vi "Calculate Curve Distance.vi"(9 "error in (no error)":errorcluster, 11 "Points":T1[](array[typedef])) -> (1 "error out":errorcluster, 2 "Length":dbl, 3 "Points Out":T1[](array[typedef]), 5 "Distance vs t":cluster{"t":dbl[], "Distance":dbl[]})   [LabVIEW 2019, in "Tool Path.lvclass"]
uses:
  Tool Path.lvclass
  Parse/PathCommands/Point.ctl
  Parse/PathCommands/PathCommands.lvclass
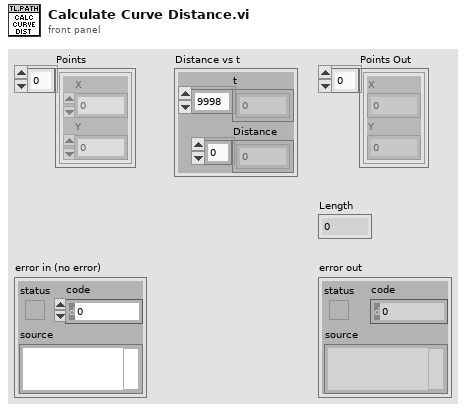
[diagram p1: front panel]
types:
  T1 = typedef "PathCommands.lvclass/Point.ctl" = cluster{"X":dbl, "Y":dbl}
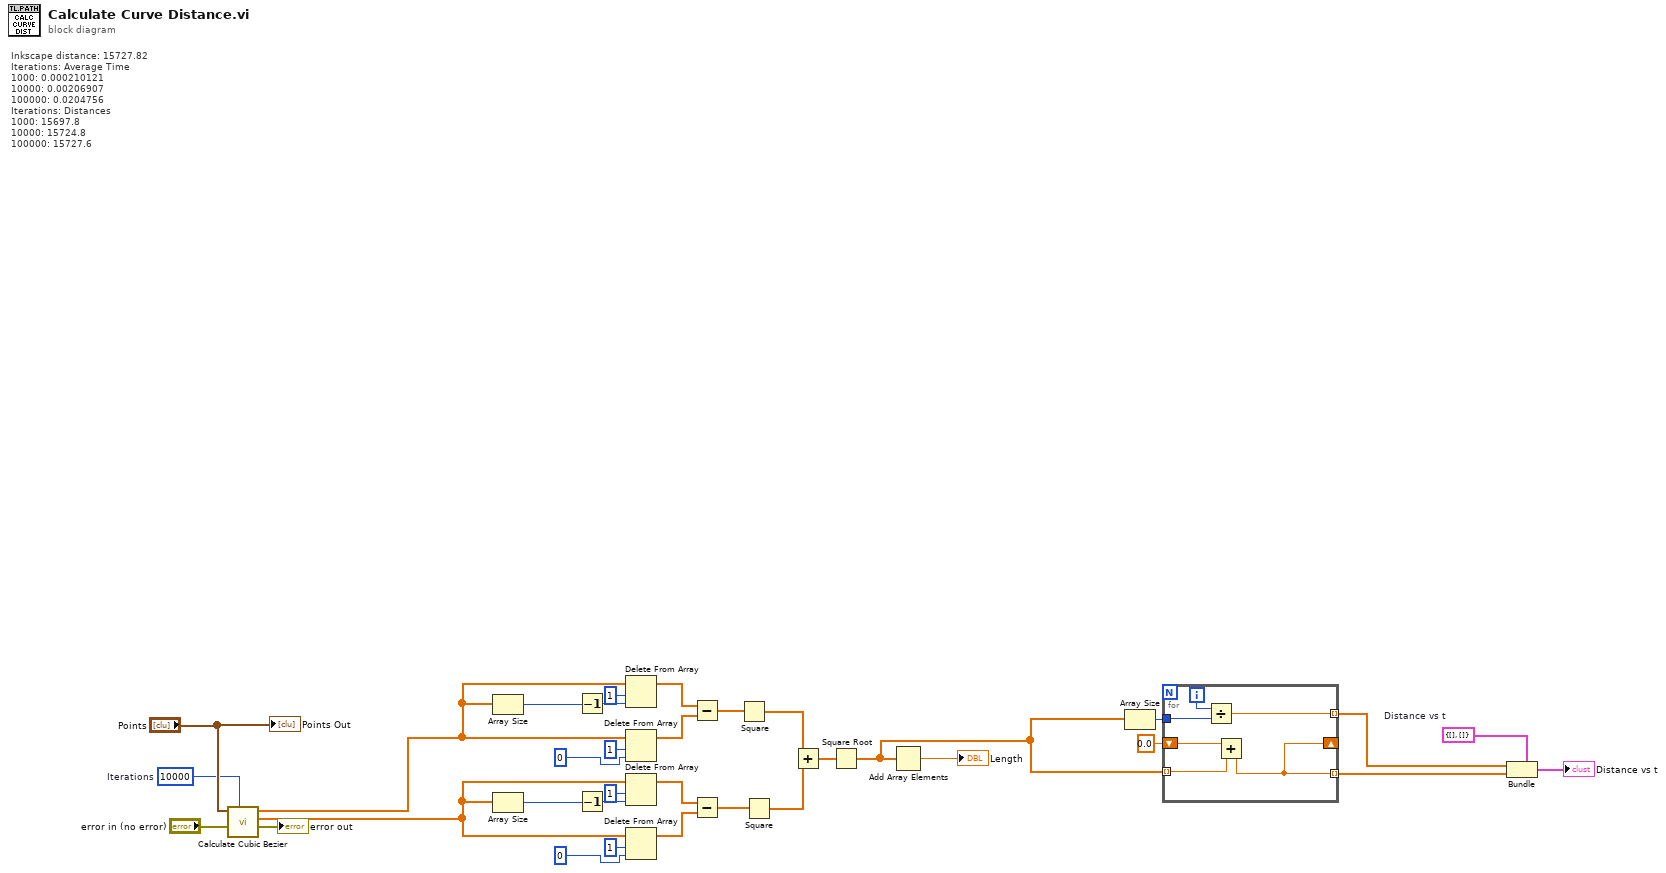
[diagram p0: block diagram]
diagram:
  w2 = cluster{"t":dbl[], "Distance":dbl[]} {"t"=[], "Distance"=[]}  # Distance vs t
  w27 = 10000  # Iterations
  # "Inkscape distance: 15727.82\nIterations: Average Time\n1000: 0.000210121\n10000: 0.00206907\n100000: 0.0204756\nIterations: Distances\n1000: 15697.8\n10000: 15724.8\n100000: 15727.6"
  n1 = call "Calculate Cubic Bezier.vi"("Iterations"=w27, "error in (no error)"="error in (no error)", "Points"="Points") -> ("error out"=→"error out":errorcluster, "Y"=w32:dbl[], "X"=w33:dbl[])  [unwired: 6 in]
  n2 = Array Size(array=w33) -> (size(s)=w13:i32)
  n3 = Array Size(array=w32) -> (size(s)=w17:i32)
  n4 = Decrement(x=w13) -> (x-1=w14:i32)
  n5 = Decrement(x=w17) -> (x-1=w16:i32)
  n6 = Delete From Array(array=w33, length=1, index=w14) -> (array with subset deleted=w21:dbl[])  [unwired: 1 out]
  n7 = Delete From Array(array=w33, length=1, index=0) -> (array with subset deleted=w22:dbl[])  [unwired: 1 out]
  n8 = Delete From Array(array=w32, length=1, index=w16) -> (array with subset deleted=w23:dbl[])  [unwired: 1 out]
  n9 = Delete From Array(array=w32, length=1, index=0) -> (array with subset deleted=w24:dbl[])  [unwired: 1 out]
  n10 = Subtract(x=w21, y=w22) -> (x-y=w15:dbl[])
  n11 = Subtract(x=w23, y=w24) -> (x-y=w18:dbl[])
  n12 = Square(x=w15) -> (x^2=w25:dbl[])
  n13 = Square(x=w18) -> (x^2=w26:dbl[])
  n14 = Add(x=w25, y=w26) -> (x+y=w19:dbl[])
  n15 = Square Root(x=w19) -> (sqrt(x)=w31:dbl[])
  n16 = Add Array Elements(numeric array=w31) -> (sum=→"Length":dbl)
  n17 = Array Size(array=w31) -> (size(s)=w3:i32)
  n18 = for {
    tunnel: w31 -> [w38] mode=indexing
    tunnel: w3 -> [w34]
    shift-right: [w36] -> _
    shift-left: 0.0 -> [w39]
    tunnel: [w36] -> w6 mode=indexing
    tunnel: [w37] -> w5 mode=indexing
    i -> [w35]
    n19 = Divide(x=w35, y=w34) -> (x/y=w37:dbl)
    n20 = Add(x=w39, y=w38) -> (x+y=w36:dbl)
  }
  n21 = Bundle(cluster=w2, "t"=w5, "Distance"=w6) -> (→"Distance vs t":cluster{"t":dbl[], "Distance":dbl[]})
  "Points Out" <- "Points"
